vi "Unicode Multilingual Interface Example.vi"() -> ()   [LabVIEW 2020]
doc: "This example demonstrates a simple multilingual interface. Translations are loaded from a unicode ini file and applied based on the selected language."
uses:
  Types/UTF-8 String/UTF-8 String.lvclass
  Unicode/Controls/String Encoding.ctl
  Types/UTF-8 String/UTF-8 String.lvclass/UTF-8 String.ctl
  Types/UTF-8 Path/UTF-8 Path.lvclass/UTF-8 Path.ctl
  <vilib>/picture/picture.llb/imagedata.ctl
  Dialog & User Interface/Message Box/Message Box Icon Type.ctl
  7a9dccd7-e3f6-4946-a880-4d7a68930416.vi
  Dialog & User Interface/Polymorphic VIs/Write Control Text/Write String Value (UTF-8 String).vi
  Dialog & User Interface/Polymorphic VIs/Write Control Text/Write Boolean Text (UTF-8 String).vi
  5a90f179-3b85-4e0c-bde1-5cde268381a4.vi
  26196076-6ab3-4cb0-b291-9633e692300f.vi
  3ad856c3-526a-4e33-8fbe-83f238f9ba6d.vi
  Unicode/Encode String.vi
  Private/Conversion/String as UTF-8 String.vi
  Private/Conversion/Polymorphic VIs/String as UTF-8 String (UTF-8 String).vi
  Dialog & User Interface/Polymorphic VIs/Write Control Text/Write String Value (UTF-8 String).vi/5206cb6b-04fb-41f5-a37e-29c14f142303.vi
  Dialog & User Interface/Polymorphic VIs/Write Control Text/Write Boolean Text (UTF-8 String).vi/5206cb6b-04fb-41f5-a37e-29c14f142303.vi
  Dialog & User Interface/Write Control Caption (Unicode).vi/13c16a8b-00d3-486b-99f0-c83eae9facb1.vi
  Private/Conversion/String as Encoded String.vi
  Private/Conversion/Polymorphic VIs/String as Encoded String (UTF-8 String).vi
  Private/Conversion/Text as Encoded String.vi
  Private/Conversion/Polymorphic VIs/Text as Encoded String (UTF-8 Path).vi
  Private/Library/gu_open_file_dialog.vi
  Private/Library/gu_select_folder_dialog.vi
  Types/UTF-8 Path/Write Encoded UTF-8 Path.vi
  26196076-6ab3-4cb0-b291-9633e692300f.vi/c24c063b-f849-48a1-b323-238a063d7118.vi
  26196076-6ab3-4cb0-b291-9633e692300f.vi/a2fd6c11-d594-45c9-8624-1f0a1df69df3.vi
  26196076-6ab3-4cb0-b291-9633e692300f.vi/1fd3173e-d32e-42cb-8f0d-819132eb8e27.vi
  26196076-6ab3-4cb0-b291-9633e692300f.vi/bb7c39fc-ad8e-447d-bc50-468674bfb562.vi
  Private/Conversion/Path as UTF-8 Path.vi
  Private/Conversion/Polymorphic VIs/Path as UTF-8 Path (UTF-8 Path).vi
  Unicode/Detect String Encoding.vi
  Private/Conversion/Text to UTF-8.vi
  Private/Conversion/Polymorphic VIs/Text to UTF-8 (LabVIEW String).vi
  Private/Conversion/Encoded UTF-8 String to Encoded UTF-16LE String.vi
  Unicode/SubVIs/UTF-16 Byte Swap.vi
  Private/Conversion/UTF-8 to Text.vi
  Private/Conversion/Polymorphic VIs/UTF-8 to Text (LabVIEW String).vi
  Private/Conversion/Encoded UTF-16LE String to Encoded UTF-8 String.vi
  Unicode/Prepend BOM.vi
  Private/Conversion/Polymorphic VIs/Text as Encoded String (UTF-8 String).vi
  Types/UTF-8 Path/Read Encoded UTF-8 Path.vi
  Private/Memory/Copy String.vi
  Private/Library/Result To Error.vi
  Private/Conversion/Path as Encoded Path.vi
  Private/Conversion/Polymorphic VIs/Path as Encoded Path (UTF-8 Path).vi
  Types/UTF-8 String/Write Encoded UTF-8 String.vi
  Private/Library/gu_string_subset.vi
  Private/Library/gu_to_lower_case.vi
  Private/Library/gu_search_split_string.vi
  Private/Conversion/Polymorphic VIs/String as Encoded String (LabVIEW String).vi
  Unicode/Strip BOM.vi
  Unicode/Detect String Encoding.vi/f4e2713d-ca87-487a-b901-d606fc3002c3.vi
  Unicode/SubVIs/Byte Order Marks.vi
  Unicode/Detect BOM.vi
  Private/Memory/Copy String.vi/4d47babd-4a2d-4eb7-b91b-7e707d692665.vi
  Private/Library/gu_free.vi
  <vilib>/Utility/config.llb/Read Key (String).vi
  Private/Library/gu_is_text_utf16.vi
  Private/Library/gu_is_text_utf8.vi
  Types/UTF-8 String/Encode UTF-8 String.vi
  Private/User Interface/Write String.vi
  Private/User Interface/Write Boolean Text.vi
  Private/User Interface/Write Caption.vi
  <vilib>/Utility/error.llb/Error Cluster From Error Code.vi
  Private/Memory/Copy String Array.vi
  Private/Library/gu_message_box.vi
  Types/UTF-8 Path/UTF-8 Path.lvclass
  <vilib>/Utility/config.llb/NI_LVConfig.lvlib
  G-Unicode.lvlib
panel:
  in  "Language":u16(ring) items=["english", "arabic", "chinese", "japanese", "korean", "polish", "russian", "thai"]
  in  "button":bool caption="¹0¤0Ã0Á0"
  out "message":string="Hello. Here is the interface in English."
  out "height":i16 caption="Height"
  out "width":i16 caption="Width"
  out "image":picture caption="Image"
  # "Instructions:\n1. Run the VI.\n2. Select a language from the text ring. The UI will update to display in that language.\n3. Click the Open File button and select an image file (note the file dialog title is also translated).\n4. The image will be loaded. If a non-image file was selected, a translated error message dialog is displayed."
  # "G"
  # "-Unicode"
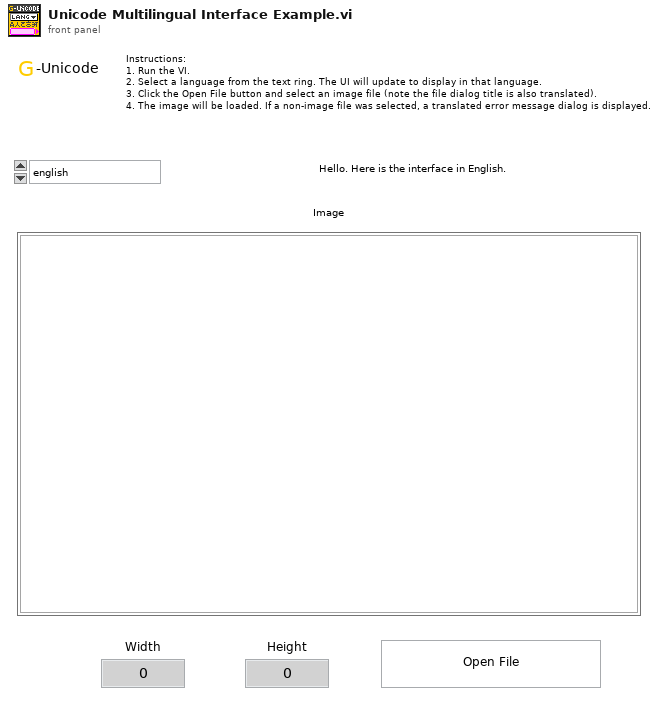
[diagram p1: front panel]
types:
  T1 = map{string, map{string, refnum<class "UTF-8 String.lvclass">}}
  T2 = typedef "NI_LVConfig.lvlib/Config Data RefNum.ctl" = refnum<k1>
  T3 = map{string, refnum<class "UTF-8 String.lvclass">}
  T4 = typedef "G-Unicode.lvlib/String Encoding.ctl" = enum16{"ANSI", "UTF-8", "UTF-16LE", "UTF-16BE", "Unknown"}
  T5 = typedef "G-Unicode.lvlib/Message Box Icon Type.ctl" = enum16{"Info", "Warning", "Error", "Question"}
  T6 = typedef "imagedata.ctl" = cluster{"image type":i32, "image depth":i32, "image":u8[], "mask":u8[], "colors":u32[], "Rectangle":cluster{"left":i16, "top":i16, "right":i16, "bottom":i16}}
  T7 = typedef "G-Unicode.lvlib/Encoded UTF-8 String.ctl" = string
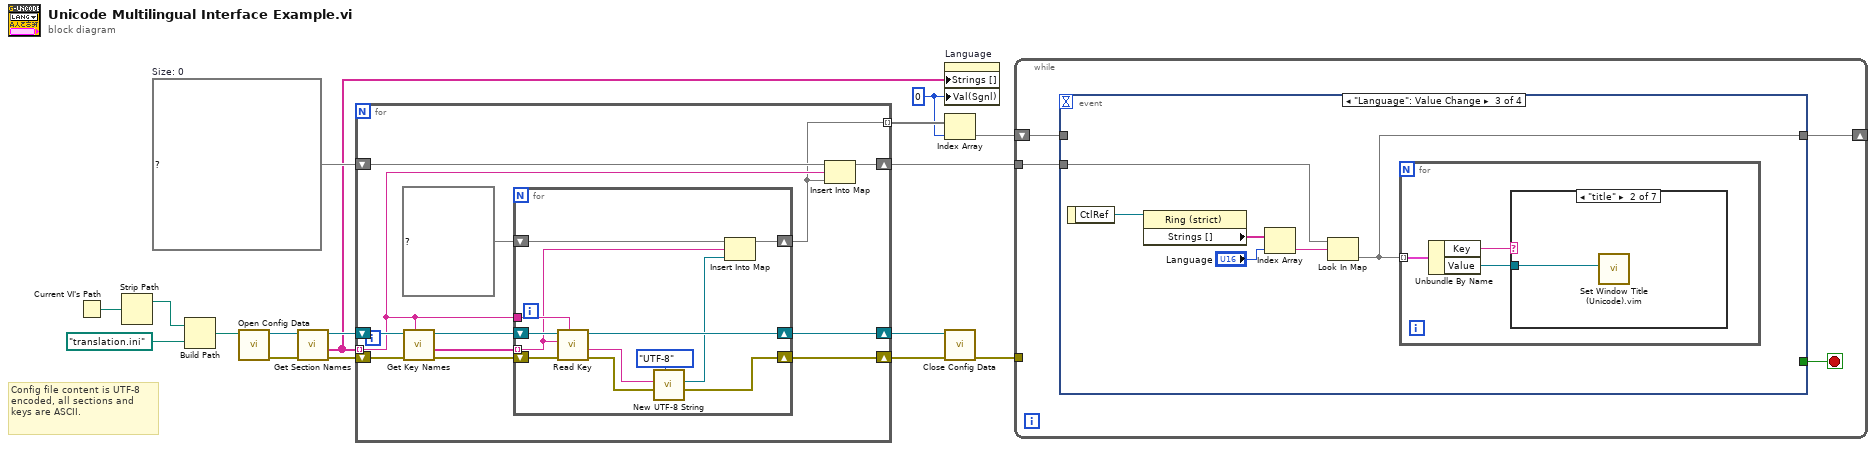
[diagram p0: block diagram]
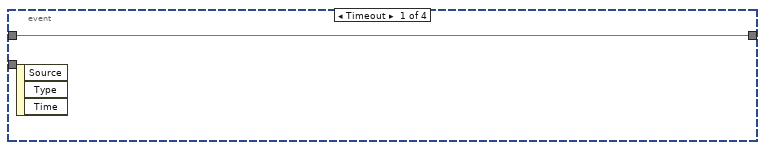
[diagram p2: hidden frame]
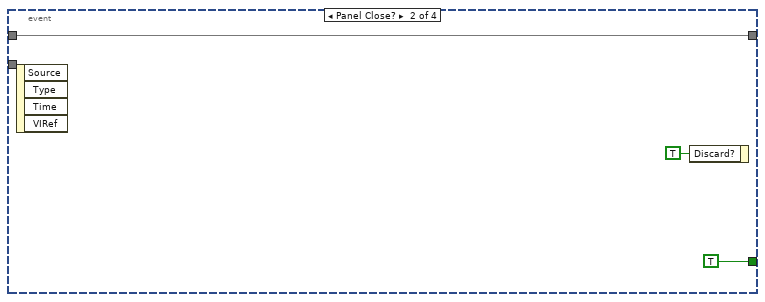
[diagram p3: hidden frame]
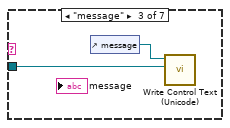
[diagram p5: hidden frame]
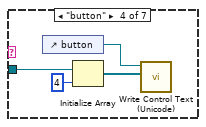
[diagram p6: hidden frame]
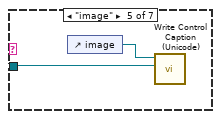
[diagram p7: hidden frame]
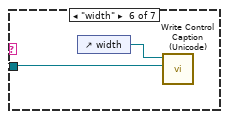
[diagram p8: hidden frame]
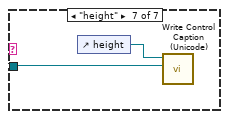
[diagram p9: hidden frame]
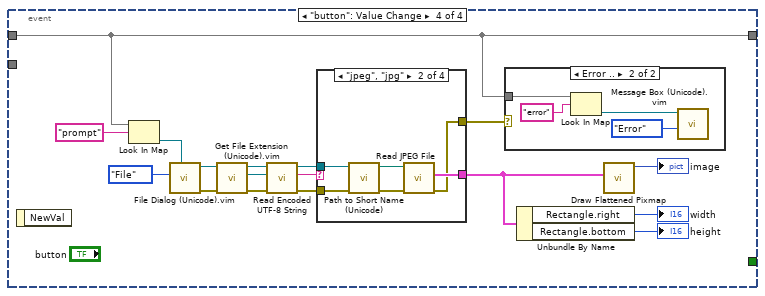
[diagram p10: hidden frame]
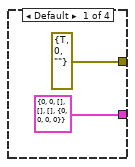
[diagram p12: hidden frame]
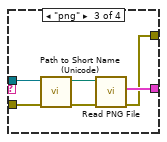
[diagram p13: hidden frame]
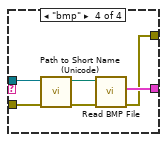
[diagram p14: hidden frame]
diagram:
  w1 = u16 0 ("Value (Signaling)")
  w11 = T1 {}  # Size: 0
  # "Config file content is UTF-8 encoded, all sections and keys are ASCII."
  n1 = Current VI's Path() -> (path=w10:path)
  n2 = Strip Path(path=w10) -> (stripped path=w8:path)  [unwired: 1 out]
  n3 = Build Path(base path=w8, name or relative path=path "translation.ini") -> (appended path=w7:path)
  n4 = call <vilib>:"Open Config Data.vi"("configuration file path"=w7) -> ("error out"=w13:errorcluster, "refnum"=w17:T2)  [unwired: 8 in, 1 out]
  n5 = call <vilib>:"Get Section Names.vi"("error in (no error)"=w13, "refnum"=w17) -> ("error out"=w14:errorcluster, "section names"=w2:string[], "refnum out"=w16:T2)  [unwired: 7 in]
  n6 = for {
    tunnel: w2 -> [w20] mode=indexing
    shift-right: [w26] -> w15
    shift-left: w16 -> [w29]
    shift-right: [w25] -> w12
    shift-left: w14 -> [w24]
    shift-right: [w22] -> w5
    shift-left: w11 -> [w21]
    tunnel: [w18] -> w3 mode=indexing
    n7 = call <vilib>:"Get Key Names.vi"("section"=w20, "error in (no error)"=w24, "refnum"=w29) -> ("error out"=w23:errorcluster, "key names"=w28:string[], "refnum out"=w27:T2)  [unwired: 5 in, 1 out]
    n8 = for {
      tunnel: w28 -> [w32] mode=indexing
      shift-right: [w40] -> w26
      shift-left: w27 -> [w41]
      tunnel: w20 -> [w38]
      shift-right: [w35] -> w25
      shift-left: w23 -> [w34]
      shift-right: [w30] -> w18
      shift-left: T3 {} ("Translation") -> [w33]
      n9 = call-poly <vilib>:"Read Key.vi"("section"=w38, "error in (no error)"=w34, "key"=w32, "refnum"=w41) -> ("error out"=w36:errorcluster, "value"=w37:string, "refnum out"=w40:T2)  [unwired: 4 in, 1 out]
      n10 = call "New UTF-8 String.vi"("Input Encoding (ANSI)"=String_Encoding."UTF-8", "error in"=w36, "String"=w37) -> ("error out"=w35:errorcluster, "UTF-8 String"=w31:refnum<class "UTF-8 String.lvclass">)  [unwired: 7 in]
      n11 = Insert Into Map(map in=w33, key=w32, value=w31) -> (map out=w30:T3)  [unwired: 2 out]
    }
    n12 = Insert Into Map(map in=w21, key=w20, value=w18) -> (map out=w22:T1)  [unwired: 2 out]
  }
  n13 = property on="Language" class="Ring (strict)"("Strings []"=w2, "Val(Sgnl)"=w1) -> ()  [unwired: 2 in, 2 out]
  n14 = Index Array(array=w3, index=w1) -> (element=w4:T3)
  n15 = call <vilib>:"Close Config Data.vi"("error in (no error)"=w12, "refnum"=w15) -> ("error out"=w6:errorcluster)  [unwired: 8 in, 1 out]
  n16 = while {
    tunnel: w5 -> [w45]
    tunnel: w6 -> [_]
    shift-right: [w44] -> _
    shift-left: w4 -> [w43]
    stop <- w42 stop-if-true
    n17 = event shown="[2] \"Language\": Value Change" {
      selector: _ -> [_ _ _ _]
      dyn-events: _ -> [_ _ _ _]
      timeout: _ -> [_ _ _ _]
      tunnel: w45 -> [_ _ w55 _]
      tunnel: [w46 w49 w51 w74] -> w44
      tunnel: w43 -> [w46 w49 _ w74]
      tunnel: [_ TRUE _ _] -> w42
      event Timeout {
        n18 = event-data() -> ()  [unwired: 1 in, 3 out]
      }
      event Panel Close? {
        n19 = event-data() -> ()  [unwired: 1 in, 4 out]
        n20 = event-data("Discard?"=TRUE) -> ()  [unwired: 1 in, 1 out]
      }
      event "Language": Value Change {
        n21 = event-data() -> ("CtlRef"=w54:refnum<vi>)  [unwired: 1 in]
        n22 = property class="Ring (strict)"(reference=w54) -> ("Strings []"=w53:string[])  [unwired: 1 in, 2 out]
        n23 = Index Array(array=w53, index="Language") -> (element=w52:string)
        n24 = Look In Map(map=w55, key=w52) -> (value=w51:T3)  [unwired: 1 in, 1 out]
        n25 = for {
          tunnel: w51 -> [w58] mode=indexing
          n26 = Unbundle By Name(w58) -> ("Key"=w57:string, "Value"=w56:refnum<class "UTF-8 String.lvclass">)
          n27 = case shown="\"title\"" w57 {
            tunnel: w56 -> [_ w59 w60 w65 w66 w69 w71]
            frame Default {
            }
            frame "title" {
              n28 = call "Set Window Title (Unicode).vim"("Title"=w59) -> ()  [unwired: 11 in]
            }
            frame "message" {
              n29 = control-ref of="message"() -> (w61:refnum<vi>)
              n30 = call-poly "Write Control Text (Unicode).vi"("Value"=w60, "Control Ref"=w61) -> ()  [unwired: 9 in, 1 out]
            }
            frame "button" {
              n31 = control-ref of="button"() -> (w62:refnum<vi>)
              n32 = Initialize Array(w65, 4 ("dimension size")) -> (w63:refnum<class "UTF-8 String.lvclass">[])
              n33 = call-poly "Write Control Text (Unicode).vi"("Value"=w63, "Control Ref"=w62) -> ()  [unwired: 9 in, 1 out]
            }
            frame "image" {
              n34 = control-ref of="image"() -> (w67:refnum<vi>)
              n35 = call "Write Control Caption (Unicode).vi"("Text"=w66, "Control Ref"=w67) -> ()  [unwired: 9 in, 1 out]
            }
            frame "width" {
              n36 = control-ref of="width"() -> (w68:refnum<vi>)
              n37 = call "Write Control Caption (Unicode).vi"("Text"=w69, "Control Ref"=w68) -> ()  [unwired: 9 in, 1 out]
            }
            frame "height" {
              n38 = control-ref of="height"() -> (w70:refnum<vi>)
              n39 = call "Write Control Caption (Unicode).vi"("Text"=w71, "Control Ref"=w70) -> ()  [unwired: 9 in, 1 out]
            }
          }
        }
      }
      event "button": Value Change {
        n40 = event-data() -> ()  [unwired: 1 in, 1 out]
        n41 = Look In Map(map=w74, key="prompt") -> (value=w75:refnum<class "UTF-8 String.lvclass">)  [unwired: 1 in, 1 out]
        n42 = call "File Dialog (Unicode).vim"("Prompt"=w75, "Selection"=enum16{"File", "Multiple Files", "Folder"}."File") -> ("error out"=w73:errorcluster, "Selected Path"=w85:refnum<class "UTF-8 Path.lvclass">)  [unwired: 6 in, 2 out]
        n43 = call "Get File Extension (Unicode).vim"("error in (no error)"=w73, "file"=w85) -> ("error out"=w72:errorcluster, "lowercase file extension"=w84:refnum<class "UTF-8 String.lvclass">, "dup file"=w82:refnum<class "UTF-8 Path.lvclass">)  [unwired: 5 in, 2 out]
        n44 = call "Read Encoded UTF-8 String.vi"("UTF-8 String"=w84) -> ("Encoded UTF-8 String"=w83:T7)  [unwired: 10 in]
        n45 = case shown="\"jpeg\", \"jpg\"" w83 {
          tunnel: w82 -> [_ w98 w104 w110]
          tunnel: [T6 {"image type"=0, "image depth"=0, "image"=[], "mask"=[], "colors"=[], "Rectangle"={"left"=0, "top"=0, "right"=0, "bottom"=0}} ("image data") w96 w102 w108] -> w80
          tunnel: [errorcluster {"status"=TRUE, "code"=0, "source"=""} ("error out") w95 w101 w107] -> w77
          tunnel: w72 -> [_ w93 w100 w106]
          frame Default {
          }
          frame "jpeg", "jpg" {
            n46 = call "Path to Short Name (Unicode).vi"("error in"=w93, "Path"=w98) -> ("error out"=w94:errorcluster, "LabVIEW Path"=w97:path)  [unwired: 8 in]
            n47 = call <vilib>:"Read JPEG File.vi"("error in (no error)"=w94, "path to JPEG file"=w97) -> ("error out"=w95:errorcluster, "image data"=w96:T6)  [unwired: 7 in, 1 out]
          }
          frame "png" {
            n48 = call "Path to Short Name (Unicode).vi"("error in"=w100, "Path"=w104) -> ("error out"=w99:errorcluster, "LabVIEW Path"=w103:path)  [unwired: 8 in]
            n49 = call <vilib>:"Read PNG File.vi"("error in (no error)"=w99, "path to PNG file"=w103) -> ("error out"=w101:errorcluster, "image data"=w102:T6)  [unwired: 7 in, 1 out]
          }
          frame "bmp" {
            n50 = call "Path to Short Name (Unicode).vi"("error in"=w106, "Path"=w110) -> ("error out"=w105:errorcluster, "LabVIEW Path"=w109:path)  [unwired: 8 in]
            n51 = call <vilib>:"Read BMP File.vi"("error in (no error)"=w105, "path to BMP file"=w109) -> ("error out"=w107:errorcluster, "image data"=w108:T6)  [unwired: 7 in, 1 out]
          }
        }
        n52 = case shown="Error .." w77 {
          tunnel: w74 -> [_ w88]
          frame No Error {
          }
          frame Error {
            n53 = Look In Map(map=w88, key="error") -> (value=w87:refnum<class "UTF-8 String.lvclass">)  [unwired: 1 in, 1 out]
            n54 = call "Message Box (Unicode).vim"("Icon (Info)"=Message_Box_Icon_Type."Error", "Message"=w87) -> ()  [unwired: 8 in, 2 out]
          }
        }
        n55 = Unbundle By Name(w80) -> ("Rectangle.right"=→"width":i16, "Rectangle.bottom"=→"height":i16)
        n56 = call <vilib>:"Draw Flattened Pixmap.vi"("image data"=w80) -> ("new picture"=→"image":picture)  [unwired: 8 in]
      }
    }
  }
